vi "Listen.vi"(8 "error in (no error)":errorcluster, 11 "CIFPlugin in":refnum<class "CAN_Reader_CANsub_Plugin.lvclass">) -> (0 "error out":errorcluster, 3 "CIFPlugin out":refnum<class "CAN_Reader_CANsub_Plugin.lvclass">)   [LabVIEW 2021, in "CAN_Reader_CANsub_Plugin.lvclass"]
uses:
  CAN_Reader_CANsub_Plugin.lvclass
  CAN_Reader_CANsub_Plugin.lvclass/CAN_Reader_CANsub_Plugin.ctl
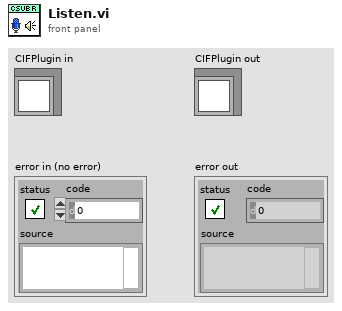
[diagram p1: front panel]
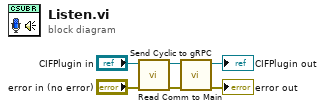
[diagram p0: block diagram]
diagram:
  n1 = call "Read Comm to Main.vi"("error in (no error)"="error in (no error)", "CIFPlugin in"="CIFPlugin in") -> ("error out"=w6:errorcluster, "CIFPlugin out"=w5:refnum<class "CAN_Reader_CANsub_Plugin.lvclass">)  [unwired: 8 in]
  n2 = call "Send Cyclic to gRPC.vi"("error in (no error)"=w6, "CIFPlugin in"=w5) -> ("error out"=→"error out":errorcluster, "CIFPlugin out"=→"CIFPlugin out":refnum<class "CAN_Reader_CANsub_Plugin.lvclass">)  [unwired: 8 in]
